vi "Get translation.vi"(7 "Type":T1=enum."String Value", 8 "error in (no error)":errorcluster, 10 "Language(\"\"=Startup Language)":string, 11 "Label":string) -> (0 "error out":errorcluster, 3 "Translation":string)   [LabVIEW 2019, in "Language Selection.lvlib"]
doc: "Returns the translation of one property of a front panel element.\n- - -\nCopyright (c) 2026, Merecs Engineering GmbH"
uses:
  Language Selection.lvlib
  TypeDefs/Enum Property Type.ctl
  <vilib>/Utility/error.llb/Trim Whitespace.vi
panel:
  out "Output 2":string
  out "Unicode?":bool
  # "Connector Pane"
  # "Locals"
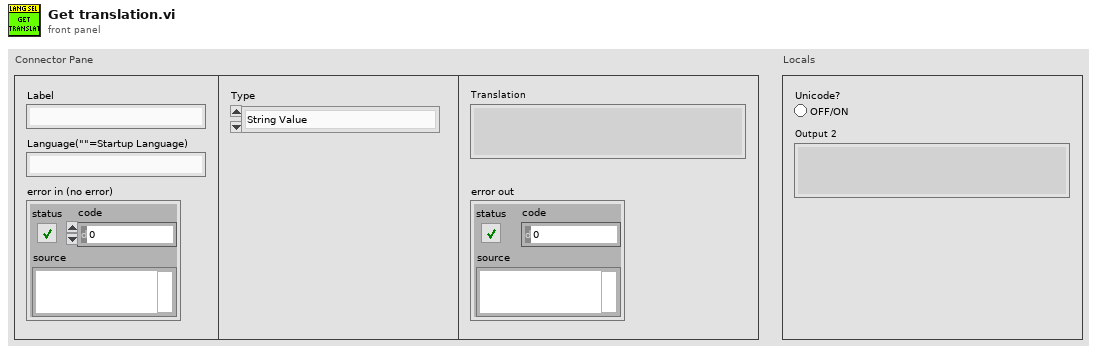
[diagram p1: front panel]
types:
  T1 = typedef "Language Selection.lvlib/Enum Property Type.ctl" = enum16{"NA", "Caption", "String Value", "Boolean Text", "Ring Strings", "1D Array Elements", "2D Array Elements", "(MC)Listbox Header", "(MC)Listbox Items", "Tab Pages Names", "X & Y GraphChart", "Plot Names", "Table Headers", "Table Items", "TipStrip", "Combobox Strings", "Cursor Name", "Tree Col Headers"}
  T2 = typedef "Language Selection.lvlib/Cluster LanguageClusterWithRefnum.ctl" = cluster{"Property":T3[], "Controls":set{refnum<vi>}}
  T3 = typedef "Language Selection.lvlib/Cluster PropertyTranslation.ctl" = cluster{"Type":T1, "Translation ANSI":string[], "Translation Unicode":string[]}
  T4 = typedef "Language Selection.lvlib/Enum Language.ctl" = i32
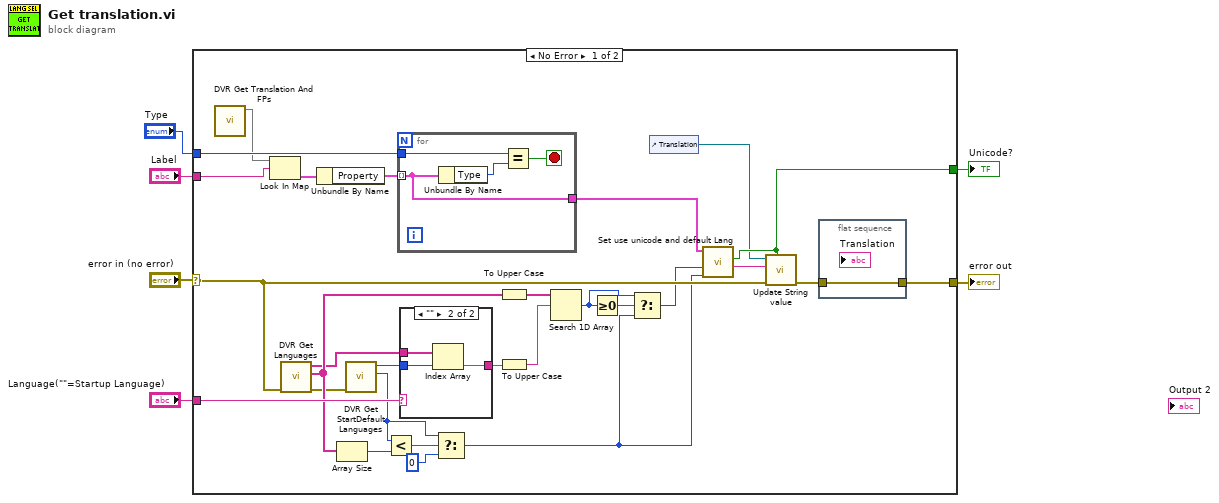
[diagram p0: block diagram]
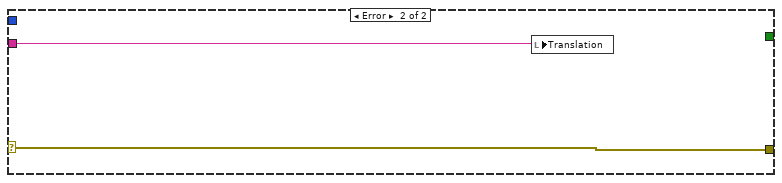
[diagram p3: hidden frame]
diagram:
  n1 = case shown="No Error" "error in (no error)" {
    selector: "error in (no error)" -> [w32 w45]
    tunnel: "Language(\"\"=Startup Language)" -> [w34 _]
    tunnel: "Label" -> [w7 w44]
    tunnel: [w33 w45] -> w6
    tunnel: [w31 _] -> w2
    tunnel: "Type" -> [w30 _]
    frame No Error {
      n2 = call "DVR Get Translation And FPs.vi"() -> ("FP Translation"=w9:map{string, T2})  [unwired: 9 in, 2 out]
      n3 = Look In Map(map=w9, key=w7) -> (value=w8:T2)  [unwired: 1 in, 1 out]
      n4 = call "DVR Get Languages.vi"("error in (no error)"=w32) -> ("error out"=w17:errorcluster, "ANSI"=w29:string[], "Languages"=w20:string[])  [unwired: 7 in, 1 out]
      n5 = Unbundle By Name(w8) -> ("Property"=w28:T3[])
      n6 = Array Size(array=w29) -> (size(s)=w24:i32)
      n7 = call "DVR Get StartDefault Languages.vi"("error in (no error)"=w17) -> ("Default"=w18:i32, "Start"=w19:T4)  [unwired: 8 in, 1 out]
      n8 = Less?(x=w18, y=w24) -> (x < y?=w23:bool)
      n9 = for {
        tunnel: w28 -> [w37] mode=indexing
        tunnel: [w37] -> w13
        tunnel: w30 -> [w38]
        stop <- w36 stop-if-true
        n10 = Unbundle By Name(w37) -> ("Type"=w39:T1)
        n11 = Equal?(x=w38, y=w39) -> (x = y?=w36:bool)
      }
      n12 = case shown="\"\"" w34 {
        selector: w34 -> [w40 _]
        tunnel: [w40 w42] -> w21
        tunnel: w20 -> [_ w43]
        tunnel: w19 -> [_ w41]
        frame Default {
        }
        frame "" {
          n13 = Index Array(array=w43, index=w41) -> (element=w42:string)
        }
      }
      n14 = Select(t=w18, s=w23, f=0 ("index")) -> (s? t:f=w15:i32)
      n15 = To Upper Case(1:w29) -> (0:w26:string[])
      n16 = To Upper Case(1:w21) -> (0:w27:string)
      n17 = Search 1D Array(1D array=w26, element=w27) -> (index of element=w16:i32)  [unwired: 1 in]
      n18 = Greater Or Equal To 0?(x=w16) -> (x >= 0?=w25:bool)
      n19 = Select(t=w16, s=w25, f=w15) -> (s? t:f=w14:i32)
      n20 = control-ref of="Translation"() -> (w10:refnum<vi>)
      n21 = call "Set use unicode and default Lang.vi"("Default Language"=w15, "Startup Language"=w14, "Obj."=w13) -> ("Translation out"=w12:string, "Unicode?"=w31:bool)  [unwired: 7 in]
      n22 = call "Update String value.vi"("Interpret as Unicode (T)"=w31, "error in (no error)"=w32, "String Value"=w12, "String Control Reference In"=w10) -> ("error out"=w11:errorcluster)  [unwired: 6 in, 1 out]
      n23 = flat-sequence {
        tunnel: [w35] -> w33
        tunnel: w11 -> [w35]
        frame #0 {
        }
      }
    }
    frame Error {
      n24 = local write "Translation"(w44) -> ()
    }
  }
  "error out" <- w6
  "Unicode?" <- w2
